vi "GpuMat ReCreate.vi"(6 "cvType":T1, 8 "error in (no error)":errorcluster, 9 "Rows":i32, 10 "Cols":i32, 11 "GpuMat in":refnum<class "GpuMat.lvclass">) -> (0 "error out":errorcluster, 3 "GpuMat out":refnum<class "GpuMat.lvclass">)   [LabVIEW 2020, in "OpenLvVision_OpenCv.lvlib" / "Cuda.lvlib" / "GpuMat.lvclass"]
doc: "Allocates new GpuMat data unless the GpuMat already has specified size and type"
uses:
  GpuMat.lvclass
  C:/Users/lukas/Documents/OpenLvVision_OpenCv/SourceCode/LabView/OpenLvVision_OpenCv/_LvHelpers/EdvrObject/EdvrObject.lvclass
  TypeDef/cvType.ctl
  _LvHelpers/EdvrObject/EdvrObject.lvclass/EdvrObject.ctl
  OpenLvVision_OpenCv.lvlib
  <vilib>/Utility/error.llb/Error Cluster From Error Code.vi
  <vilib>/ErrorRing/Error Ring.xnode
  _LvHelpers/EdvrObject/EdvrObject.lvclass
  Dlls/OlvOpenCvWrapper.dll
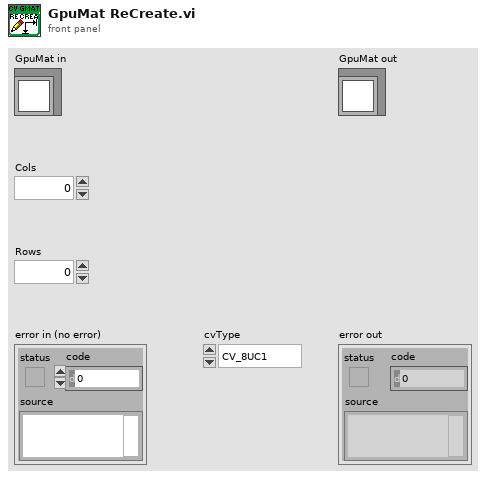
[diagram p1: front panel]
types:
  T1 = typedef "OpenLvVision_OpenCv.lvlib/cvType.ctl" = enum32{"CV_8UC1", "CV_8SC1", "CV_16UC1", "CV_16SC1", "CV_32SC1", "CV_32FC1", "CV_64FC1", "CV_16FC1", "CV_8UC2", "CV_8SC2", "CV_16UC2", "CV_16SC2", "CV_32SC2", "CV_32FC2", "CV_64FC2", "CV_16FC2", "CV_8UC3", "CV_8SC3", "CV_16UC3", "CV_16SC3", "CV_32SC3", "CV_32FC3", "CV_64FC3", "CV_16FC3", "CV_8UC4", "CV_8SC4", "CV_16UC4", "CV_16SC4", "CV_32SC4", "CV_32FC4", "CV_64FC4", "CV_16FC4"}
  T2 = typedef "OpenLvVision_OpenCv.lvlib/EdvrObject.lvclass/Edvr.ctl" = refnum<data-value>
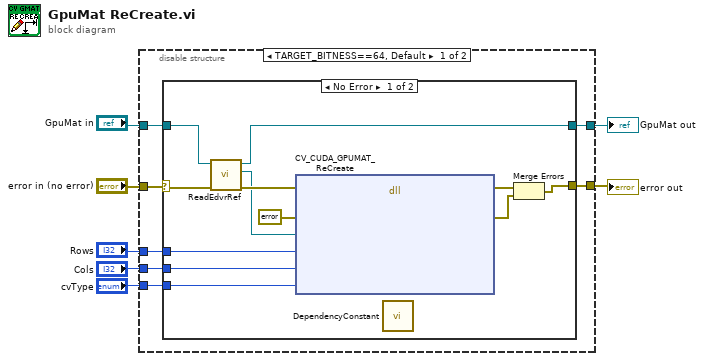
[diagram p0: block diagram]
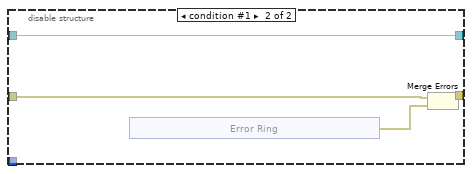
[diagram p3: hidden frame]
diagram:
  n1 = disable-structure shown="TARGET_BITNESS==64, Default" {
    disable-tunnel: "error in (no error)" -> [w14 w31]
    disable-tunnel: [w13 w32] -> w7
    disable-tunnel: "GpuMat in" -> [w12 w29]
    disable-tunnel: [w11 w29] -> w4
    disable-tunnel: "Rows" -> [w10 _]
    disable-tunnel: "Cols" -> [w9 _]
    disable-tunnel: "cvType" -> [w8 _]
    frame condition #0 (active) {
      n2 = case shown="No Error" w14 {
        selector: w14 -> [w18 w28]
        tunnel: [w23 w28] -> w13
        tunnel: w12 -> [w21 w27]
        tunnel: [w19 w27] -> w11
        tunnel: w10 -> [w17 _]
        tunnel: w9 -> [w16 _]
        tunnel: w8 -> [w15 _]
        frame No Error {
          n3 = call "ReadEdvrRef.vi"("error in (no error)"=w18, "EdvrObject in"=w21) -> ("error out"=w22:errorcluster, "Edvr"=w20:T2, "EdvrObject out"=w19:refnum<class "GpuMat.lvclass">)  [unwired: 7 in]
          n4 = dll-call lib="C:/Users/lukas/Documents/OpenLvVision_OpenCv/SourceCode/LabView/OpenLvVision_OpenCv/Dlls/OlvOpenCvWrapper.dll" fn="CV_CUDA_GPUMAT_ReCreate"(error in=w22, "Error"=errorcluster {"status"=FALSE, "code"=0, "source"=""} ("error out"), "edvrRef"=w20, "rows"=w17, "cols"=w16, "cvType"=w15) -> (error out=w26:errorcluster, "Error"=w25:errorcluster)  [unwired: 7 in, 1 out]
          n5 = call "DependencyConstant.vi"() -> ()  [unwired: 12 in]
          n6 = Merge Errors(w26, w25) -> (w23:errorcluster)
        }
        frame Error {
        }
      }
    }
    frame condition #1 {
      n7 = xnode "Error Ring"() -> ("error out"=w30:errorcluster)
      n8 = Merge Errors(w31, w30) -> (w32:errorcluster)
    }
  }
  "error out" <- w7
  "GpuMat out" <- w4
